vi "lvpm Pilots.vi"(8 "error in":errorcluster, 9 "settings path":path, 10 "settings":cluster{"rate (Hz)":dbl, "channel":string}, 11 "message":string) -> (0 "error out":errorcluster, 3 "settings text":string)   [LabVIEW 2026]
doc: "Pilot helper that exercises two lvpm packages. Logs message at INFO through HSE Logger (a file handler in the temp folder named lvpm Pilots.log is created and closed in this VI) and serializes settings with OpenSerializer's PlainText serializer. Returns that PlainText as settings text and writes it to settings path when that path is not empty. Errors flow from error in through logging and the file write to error out."
uses:
  <vilib>/Hampel Software Engineering/HSE Logger/Handler/FileHandler/FileHandler.lvclass
  <vilib>/Hampel Software Engineering/HSE Logger/hse-logger.lvlib
  <vilib>/LabVIEW Open Source Project/OpenSerializer/Serializer.PlainText/Serializer.PlainText.lvclass
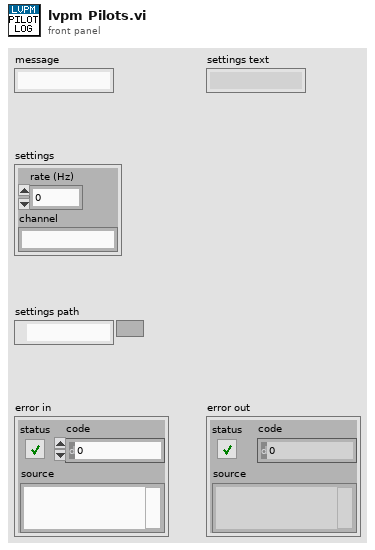
[diagram p1: front panel]
types:
  T1 = enum16{"DEBUG", "INFO", "WARNING", "ERROR", "CRITICAL"}
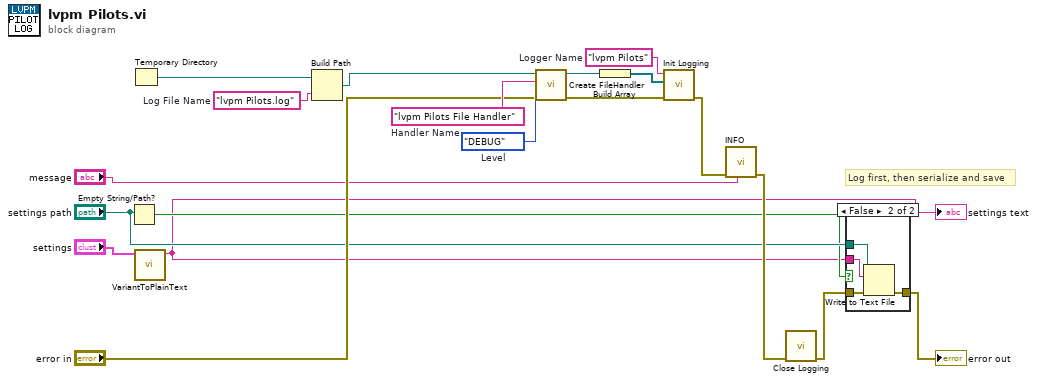
[diagram p0: block diagram]
diagram:
  w15 = T1."DEBUG"  # Level
  w18 = "lvpm Pilots.log"  # Log File Name
  w16 = "lvpm Pilots File Handler"  # Handler Name
  w12 = "lvpm Pilots"  # Logger Name
  # "Log first, then serialize and save"
  n1 = Empty String/Path?(string/path="settings path") -> (empty?=w3:bool)
  n2 = Temporary Directory() -> (w19:path)
  n3 = call <vilib>:"VariantToPlainText.vi"("Variant-formatted Value"="settings") -> ("String-formatted Value"=w2:string)  [unwired: 10 in]
  "settings text" <- w2
  n4 = Build Path(base path=w19, name or relative path=w18) -> (appended path=w17:path)
  n5 = call <vilib>:"Create FileHandler.vi"("error in"="error in", "Level"=w15, "Name"=w16, "Filepath"=w17) -> ("error out"=w10:errorcluster, "FileHandler out"=w13:refnum<class "FileHandler.lvclass">)  [unwired: 6 in]
  n6 = Build Array(w13) -> (w11:refnum<class "FileHandler.lvclass">[])
  n7 = call <vilib>:"Init Logging.vi"("error in"=w10, "Handlers"=w11, "Name"=w12) -> ("error out"=w9:errorcluster)  [unwired: 8 in]
  n8 = call <vilib>:"INFO.vi"("Message"="message", "error in"=w9) -> ("error out"=w7:errorcluster)  [unwired: 9 in]
  n9 = call <vilib>:"Close Logging.vi"("error in"=w7) -> ("error out"=w5:errorcluster)  [unwired: 10 in]
  n10 = case shown="False" w3 {
    tunnel: w5 -> [w20 w22]
    tunnel: "settings path" -> [_ w24]
    tunnel: w2 -> [_ w23]
    tunnel: [w20 w21] -> w1
    frame True {
    }
    frame False {
      n11 = Write to Text File(file (use dialog)=w24, text=w23, error in=w22) -> (error out=w21:errorcluster)  [unwired: 1 in, 2 out]
    }
  }
  "error out" <- w1
